vi "I2C Bus Monitor Test.vi"() -> ()   [LabVIEW 2025]
uses:
  b35e104c-1675-4f6f-8f1c-29597b7e93d1.vi
  I2C Bus Monitor UI/I2C Bus Monitor UI.lvlib
  I2C Bus Monitor/I2C Bus Monitor.lvclass
panel:
  in  "Complex Serdes Scripts":bool
  in  "Scan Serial Channel":string(combo)
  out "Scan Bus Error":errorcluster
  out "Scanned Addresses":i32[](array[numeric]) format="%.0x"
  in  "Scan":bool
  out "# Txns in Table":i32
  in  "Select 2":bool
  in  "SERIAL INPUT (SI)":u32(ring)
  in  "Select":bool
  in  "RESOURCE NAME":u32(ring)
  in  "I2C Scrpit Path":path
  in  "Serial Channel":string(combo)
  in  "Send I2C Script":bool
  out "I2C Script Error":errorcluster
  out "I2C Transaction Error":errorcluster
  in  "I2C Command":T1 {"Data" format="%02x"; "Register Address" format="%04x"; "Slave Address" format="%02x"}
  out "Read Data":u8 format="%02x"
  in  "Send I2C Transaction":bool
  out "User Timestamp Fifo Overflow":bool
  out "i":i32
  out "I2C Messages":string[][](table)
  out "Total Messages":i32
  out "FIFO Pressure":u32
  in  "stop":bool
  out "Bitfile Path":path
  out "SI Count":i32
  out "Module Name":string
  out "error out":errorcluster
  # "takes few seconds to populate RESOURCE NAME"
  # "1"
  # "takes few seconds to populate SERIAL INPUT (SI)"
  # "2"
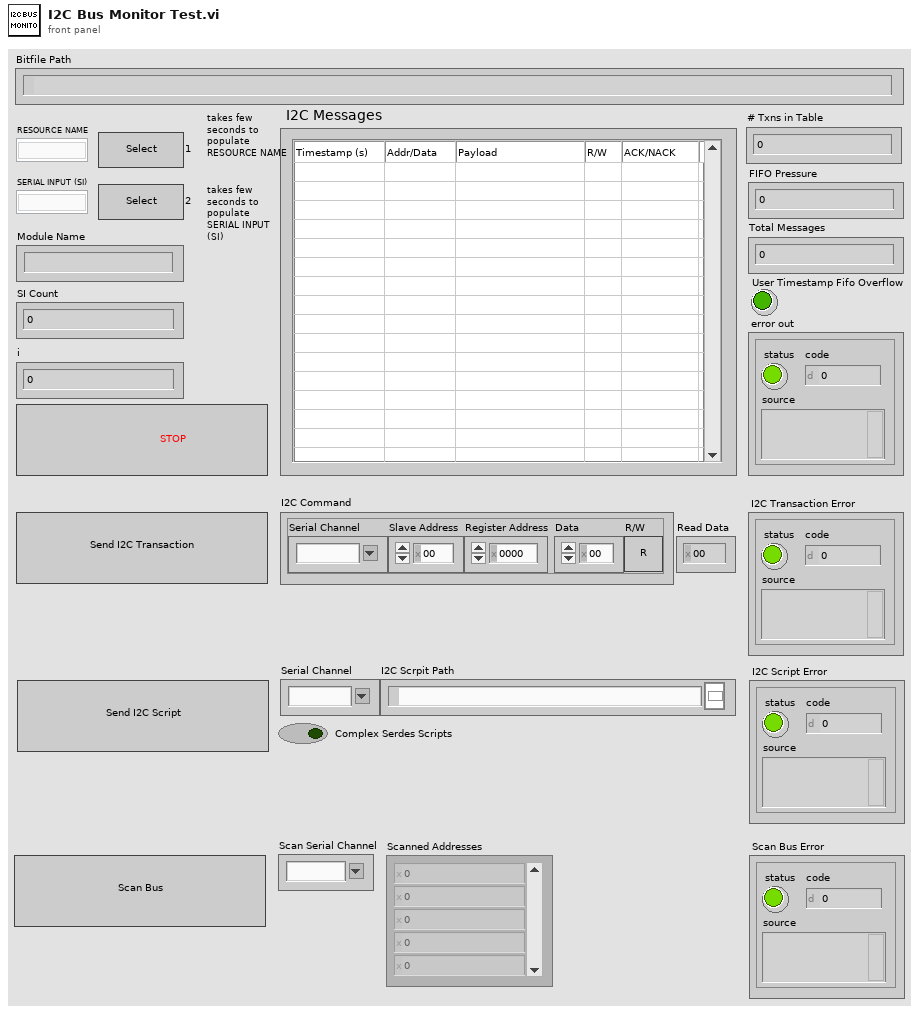
[diagram p1: front panel]
types:
  T1 = cluster{"Serial Channel":string, "Slave Address":u8, "Register Address":u16, "Data":u8, "R/W":bool}
  T2 = typedef "NI CSI-2 API FPGA v2.lvlib/Timestamp ID.ctl" = enum8{"SI0 LLP", "SI1 LLP", "SI2 LLP", "SI3 LLP", "SI4 LLP", "SI5 LLP", "SI6 LLP", "SI7 LLP", "SO0 LLP", "SO1 LLP", "SO2 LLP", "SO3 LLP", "SO4 LLP", "SO5 LLP", "SO6 LLP", "SO7 LLP", "Ser0 GPIO Bank", "Ser1 GPIO Bank", "Ser2 GPIO Bank", "Ser3 GPIO Bank", "Ser4 GPIO Bank", "Ser5 GPIO Bank", "Ser6 GPIO Bank", "Ser7 GPIO Bank", "Des0 GPIO Bank", "Des1 GPIO Bank", "Des2 GPIO Bank", "Des3 GPIO Bank", "Des4 GPIO Bank", "Des5 GPIO Bank", "Des6 GPIO Bank", "Des7 GPIO Bank", "User0", "User1", "User2", "User3", "User4", "User5", "User6", "User7", "User8", "User9", "User10", "User11", "User12", "User13", "User14", "User15", "User16", "User17", "User18", "User19", "User20", "User21", "User22", "User23", "User24", "User25", "User26", "User27", "User28", "User29", "User30", "User31"}
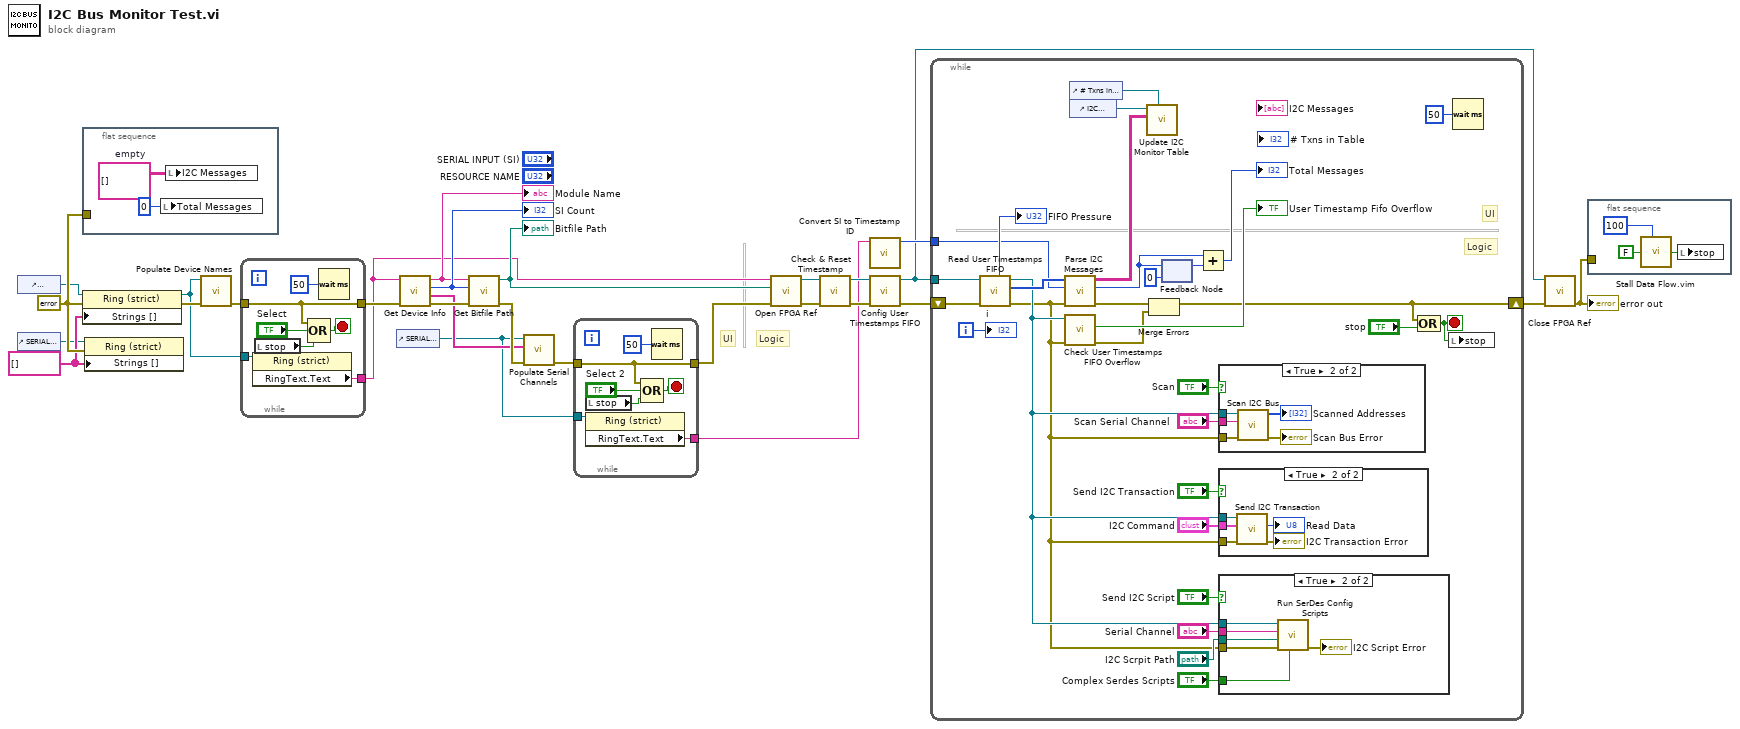
[diagram p0: block diagram]
diagram:
  w4 = string[] [] ("Strings []")
  w28 = errorcluster {"status"=FALSE, "code"=0, "source"=""} ("error constant")
  # "Logic"
  # "UI"
  n1 = control-ref of="RESOURCE NAME"() -> (w6:refnum<vi>)
  n2 = control-ref of="SERIAL INPUT (SI)"() -> (w3:refnum<vi>)
  n3 = flat-sequence {
    tunnel: w28 -> [_]
    frame #0 {
      w30 = string[][] []  # empty
      n4 = local write "Total Messages"(0 ("Total Records out")) -> ()
      n5 = local write "I2C Messages"(w30) -> ()
    }
  }
  n6 = property class="Ring (strict)"(reference=w6, error in=w28, "Strings []"=w4) -> (reference out=w5:refnum<vi>, error out=w7:errorcluster)
  n7 = property class="Ring (strict)"(reference=w3, error in=w28, "Strings []"=w4) -> ()  [unwired: 2 out]
  n8 = call "Populate Device Names.vi"("error in (no error)"=w7, "RESOURCE NAME Ref"=w5) -> ("error out"=w16:errorcluster)  [unwired: 8 in, 1 out]
  n9 = while {
    tunnel: [w34] -> w17
    tunnel: w16 -> [w34]
    tunnel: w5 -> [w33]
    tunnel: [w32] -> w8
    stop <- w35 stop-if-true
    n10 = property class="Ring (strict)"(reference=w33) -> ("RingText.Text"=w32:string)  [unwired: 1 in, 2 out]
    n11 = local read "stop"() -> (w31:bool)
    n12 = Compound Arithmetic op=OR(w34, "Select", w31) -> (w35:bool)
    n13 = Wait (ms)(milliseconds to wait=u32 50) -> ()  [unwired: 1 out]
  }
  n14 = control-ref of="SERIAL INPUT (SI)"() -> (w11:refnum<vi>)
  n15 = call "Get Device Info.vi"("error in (no error)"=w17, "RIO Device"=w8) -> ("error out"=w27:errorcluster, "SI Channels"=w14:string[], "SI Count"=w26:i32, "Module Name"=w15:string)  [unwired: 6 in]
  "Module Name" <- w15
  "SI Count" <- w26
  n16 = call "Get Bitfile Path.vi"("error in (no error)"=w27, "SI Count"=w26, "Module Name"=w15) -> ("error out"=w22:errorcluster, "Bitfile Path"=w25:path)  [unwired: 7 in]
  "Bitfile Path" <- w25
  n17 = call "Populate Serial Channels.vi"("error in (no error)"=w22, "Strings []"=w14, "SERIAL INPUT (SI) Ref in"=w11) -> ("error out"=w13:errorcluster)  [unwired: 7 in, 1 out]
  n18 = while {
    tunnel: [w42] -> w12
    tunnel: w13 -> [w42]
    tunnel: w11 -> [w41]
    tunnel: [w40] -> w9
    stop <- w43 stop-if-true
    n19 = local read "stop"() -> (w38:bool)
    n20 = property class="Ring (strict)"(reference=w41) -> ("RingText.Text"=w40:string)  [unwired: 1 in, 2 out]
    n21 = Compound Arithmetic op=OR(w42, "Select 2", w38) -> (w43:bool)
    n22 = Wait (ms)(milliseconds to wait=u32 50) -> ()  [unwired: 1 out]
  }
  n23 = call "Open FPGA Ref.vi"("error in (no error)"=w12, "Bitfile Path"=w25, "Device address"=w8) -> ("error out"=w24:errorcluster, "FPGA Ref out"=w19:refnum<k20>)  [unwired: 7 in]
  n24 = call "Check & Reset Timestamp.vi"("error in (no error)"=w24, "FPGA Ref in"=w19) -> ("error out"=w20:errorcluster, "FPGA Ref out"=w18:refnum<k20>)  [unwired: 8 in]
  n25 = call "Convert SI to Timestamp ID.vi"("SI Channel"=w9) -> ("Timestamp ID"=w21:T2)  [unwired: 10 in]
  n26 = call "Config User Timestamps FIFO.vi"("error in (no error)"=w20, "FPGA Ref in"=w18) -> ("error out"=w2:errorcluster, "FPGA Ref out"=w1:refnum<k20>)  [unwired: 8 in]
  n27 = while {
    shift-right: [w63] -> w23
    shift-left: w2 -> [w72]
    tunnel: w21 -> [w60]
    tunnel: w1 -> [w73]
    i -> [w71]
    stop <- w61 stop-if-true
    # "Logic"
    # "UI"
    n28 = call "Read User Timestamps FIFO.vi"("error in (no error)"=w72, "FPGA Ref in"=w73) -> ("error out"=w46:errorcluster, "Data"=w66:u64[], "FPGA Ref out"=w47:refnum<k20>, "Elements Remaining"=→"FIFO Pressure":u32)  [unwired: 6 in]
    n29 = call "Parse I2C Messages.vi"("error in (no error)"=w46, "Timestamp ID"=w60, "User Timestamps"=w66) -> ("error out"=w65:errorcluster, "Count"=w57:i32, "I2C Messages"=w62:string[][])  [unwired: 6 in]
    n30 = call "Check User Timestamps FIFO Overflow.vi"("error in (no error)"=w46, "FPGA Ref in"=w47) -> ("error out"=w64:errorcluster, "User Timestamp FIFO Overflow"=→"User Timestamp Fifo Overflow":bool)  [unwired: 7 in, 1 out]
    n31 = control-ref of="# Txns in Table"() -> (w53:refnum<vi>)
    n32 = control-ref of="I2C Messages"() -> (w67:refnum<vi>)
    n33 = call "Update I2C Monitor Table.vi"("# TXNS IN TABLE Ref"=w53, "I2C Data in"=w62, "I2C Table Ref"=w67) -> ()  [unwired: 8 in, 1 out]
    n34 = Merge Errors(w65, w64) -> (w63:errorcluster)
    n35 = feedback-in #1(w57) -> ()
    n36 = feedback #1(0 ("Count")) -> (w58:i32)
    n37 = Add(x=w57, y=w58) -> (x+y=→"Total Messages":i32)
    n38 = case shown="True" "Scan" {
      tunnel: w46 -> [_ w90]
      tunnel: w47 -> [_ w89]
      tunnel: "Scan Serial Channel" -> [_ w87]
      frame False {
      }
      frame True {
        n39 = call "Scan I2C Bus.vi"("error in (no error)"=w90, "Serial Input"=w87, "FPGA Ref"=w89) -> ("error out"=→"Scan Bus Error":errorcluster, "Scanned Addresses"=→"Scanned Addresses":i32[])  [unwired: 7 in]
      }
    }
    n40 = case shown="True" "Send I2C Transaction" {
      tunnel: w46 -> [_ w85]
      tunnel: "I2C Command" -> [_ w84]
      tunnel: w47 -> [_ w82]
      frame False {
      }
      frame True {
        n41 = call "Send I2C Transaction.vi"("Error In"=w85, "I2C Command"=w84, "FPGA Ref in"=w82) -> ("Error Out"=→"I2C Transaction Error":errorcluster, "Read Data"=→"Read Data":u8)  [unwired: 6 in, 1 out]
      }
    }
    n42 = case shown="True" "Send I2C Script" {
      tunnel: w46 -> [_ w80]
      tunnel: w47 -> [_ w79]
      tunnel: "I2C Scrpit Path" -> [_ w77]
      tunnel: "Serial Channel" -> [_ w76]
      tunnel: "Complex Serdes Scripts" -> [_ w75]
      frame False {
      }
      frame True {
        n43 = call "Run SerDes Config Scripts.vi"("Complex Serdes Scripts"=w75, "error in (no error)"=w80, "configuration scripts"=w77, "serial channels"=w76, "FPGA Ref In"=w79) -> ("error out"=→"I2C Script Error":errorcluster)  [unwired: 4 in, 2 out]
      }
    }
    n44 = Compound Arithmetic op=OR(w63, "stop") -> (w61:bool)
    n45 = local write "stop"(w61) -> ()
    n46 = Wait (ms)(milliseconds to wait=u32 50) -> ()  [unwired: 1 out]
    "i" <- w71
  }
  n47 = call "Close FPGA Ref.vi"("error in (no error)"=w23, "FPGA Ref in"=w1) -> ("error out"=w10:errorcluster)  [unwired: 9 in]
  "error out" <- w10
  n48 = flat-sequence {
    tunnel: w10 -> [_]
    frame #0 {
      n49 = call "Stall Data Flow.vim"("value in"=FALSE ("stop"), "milliseconds to wait"=u32 100) -> ("value out"=w92:bool)  [unwired: 1 out]
      n50 = local write "stop"(w92) -> ()
    }
  }
